vi "Update Inputs.vi"(8 "error in (no error)":errorcluster, 10 "Inputs":T1[](array[typedef]), 11 "UI Template in":refnum<class "DIO_Panel.lvclass">) -> (0 "error out":errorcluster, 3 "UI Template out":refnum<class "DIO_Panel.lvclass">)   [LabVIEW 2021, in "Simulator-Channel.lvlib" / "DIO_Panel.lvlib" / "DIO_Panel.lvclass"]
uses:
  DIO_Panel.lvclass
  tdef/info.ctl
  DIO_Panel.lvclass/DIO_Panel.ctl
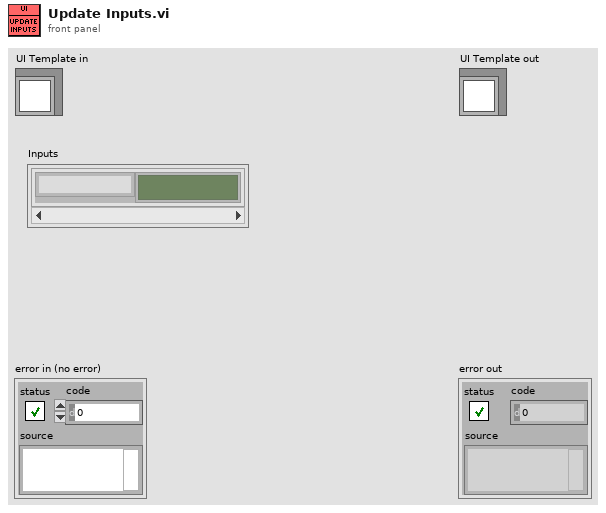
[diagram p1: front panel]
types:
  T1 = typedef "Simulator-Channel.lvlib/DIO_Panel.lvlib/DIO_Panel.lvclass/info.ctl" = cluster{"Name":string, "Boolean":bool}
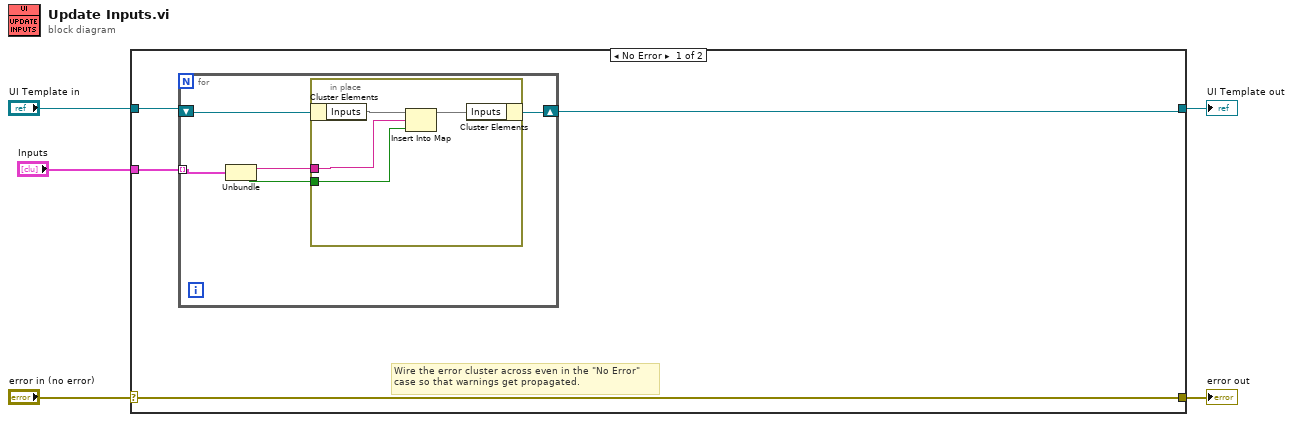
[diagram p0: block diagram]
diagram:
  n1 = case shown="No Error" "error in (no error)" {
    selector: "error in (no error)" -> [w9 w20]
    tunnel: [w9 w20] -> w4
    tunnel: [w6 w19] -> w2
    tunnel: "UI Template in" -> [w7 w19]
    tunnel: "Inputs" -> [w8 _]
    frame No Error {
      # "Wire the error cluster across even in the \"No Error\"\ncase so that warnings get propagated."
      n2 = for {
        tunnel: w8 -> [w12] mode=indexing
        shift-right: [w13] -> w6
        shift-left: w7 -> [w14]
        n3 = Unbundle(w12) -> ("Name"=w11:string, "Boolean"=w10:bool)
        n4 = in-place {
          in-place-border: w11 -> [w16]
          in-place-border: w10 -> [w15]
          n5 = in-place-cluster #1(w14) -> ("Inputs"=w18:map{string, bool})
          n6 = Insert Into Map(map in=w18, key=w16, value=w15) -> (map out=w17:map{string, bool})  [unwired: 2 out]
          n7 = in-place-cluster #1("Inputs"=w17) -> (w13:refnum<class "DIO_Panel.lvclass">)
        }
      }
    }
    frame Error {
    }
  }
  "error out" <- w4
  "UI Template out" <- w2
